vi "Destruct.vi"(8 "error in (no error)":errorcluster) -> (0 "error out":errorcluster)   [LabVIEW 2020, in "Tag Engine Core.lvlib" / "Tag Core.lvclass"]
doc: "_SubVI_"
uses:
  Tag Core.lvclass
  Tag/Tag.lvclass
  Tag/Tag.lvclass/Tag.ctl
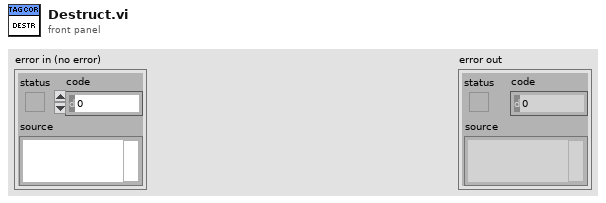
[diagram p1: front panel]
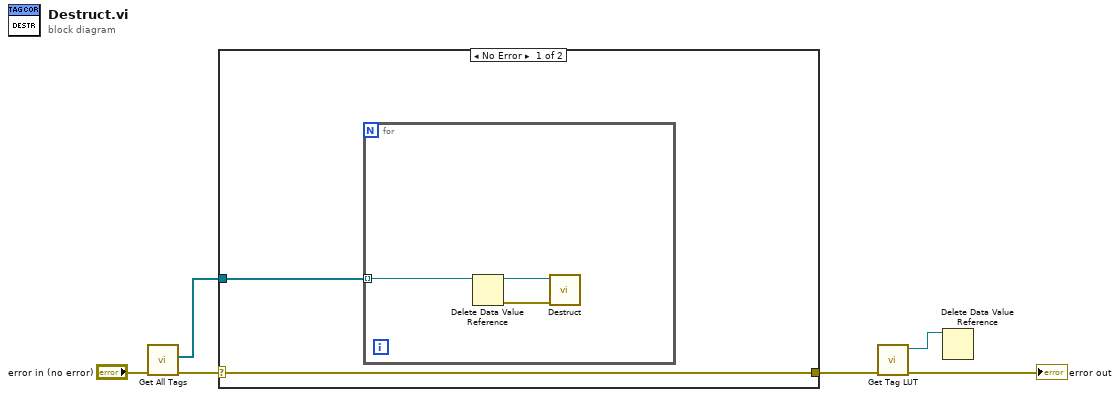
[diagram p0: block diagram]
diagram:
  n1 = call "Get All Tags.vi"("error in (no error)"="error in (no error)") -> ("error out"=w2:errorcluster, "Tag Refs"=w1:refnum<data-value>[])  [unwired: 9 in]
  n2 = case shown="No Error" w2 {
    selector: w2 -> [w8 w12]
    tunnel: [w8 w12] -> w6
    tunnel: w1 -> [w7 _]
    frame No Error {
      n3 = for {
        tunnel: w7 -> [w11] mode=indexing
        n4 = Delete Data Value Reference(data value reference=w11) -> (data value=w10:refnum<class "Tag.lvclass">, error out=w9:errorcluster)  [unwired: 1 in]
        n5 = call "Destruct.vi"("error in (no error)"=w9, "Tag in"=w10) -> ()  [unwired: 9 in, 1 out]
      }
    }
    frame Error {
    }
  }
  n6 = call "Get Tag LUT.vi"("error in (no error)"=w6) -> ("error out"=→"error out":errorcluster, "Tag LUT Out"=w5:refnum<data-value>)  [unwired: 9 in]
  n7 = Delete Data Value Reference(data value reference=w5) -> ()  [unwired: 1 in, 2 out]
